vi "LabVIEW.Service.JSON_Input.vi"(4 "Value 4":string="\"Test\"", 6 "Value 3":string="\"Test\"", 7 "Command":T1, 8 "Fehler (Eingang, kein Fehler)":errorcluster, 9 "Value[]":string[](array[string]), 10 "Value 1":string="\"Test\"", 11 "Value 2":string="\"Test\"") -> (0 "Fehler (Ausgang)":errorcluster, 3 "<JSON>":string)   [LabVIEW 2026]
uses:
  LabVIEW.Type Definitions/LabVIEW.Service.JSON_Input_Command.ctl
  <vilib>/JDP Science/JSONtext/support/Format JSON Object.vi
  <vilib>/JDP Science/JSONtext/support/Format JSON Array Text.vi
  <vilib>/JDP Science/JSONtext/JSONtext.lvlib
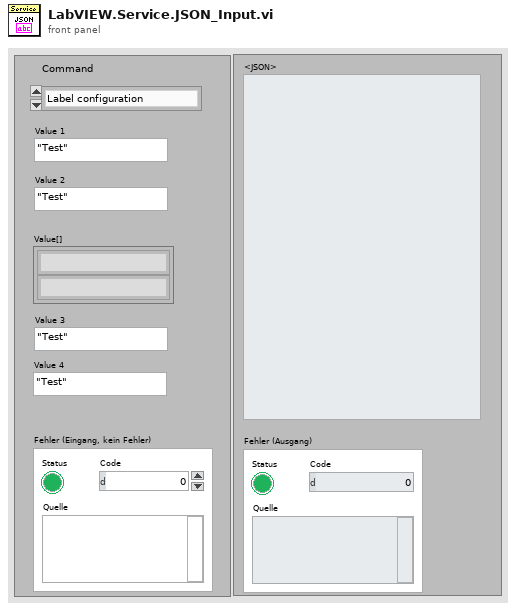
[diagram p1: front panel]
types:
  T1 = typedef "LabVIEW.Service.JSON_Input_Command.ctl" = enum16{"Label configuration", "Label colour ribbon/label tape", "Serial number info text", "Serial number update step", "Serial number bulk lookup", "Vorgang migrate serial numbers to Vorgang", "Vorgang migrate serial numbers to product revision", "Vorgang Update step states", "Fertigmeldung Create/Revert a Fertigmeldung", "User Update a user", "User Update a user role", "Create a new product", "Update a product's data"}
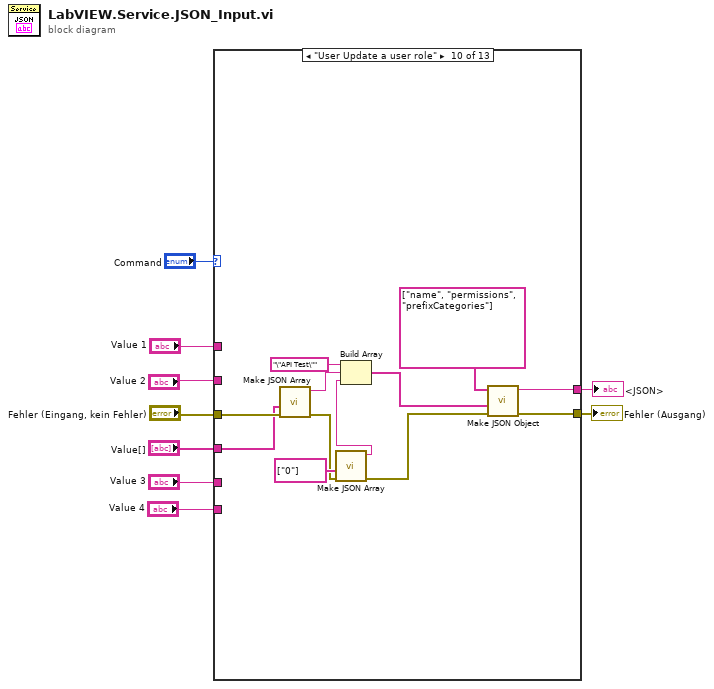
[diagram p0: block diagram]
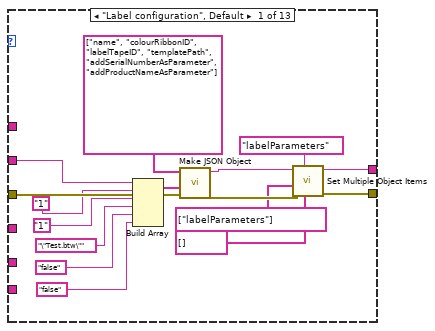
[diagram p2: hidden frame]
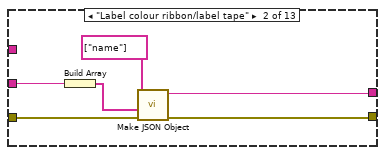
[diagram p3: hidden frame]
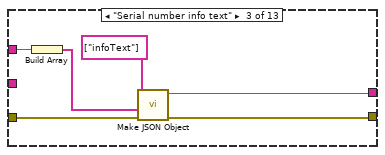
[diagram p4: hidden frame]
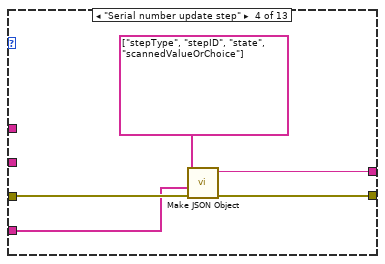
[diagram p5: hidden frame]
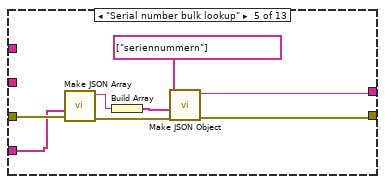
[diagram p6: hidden frame]
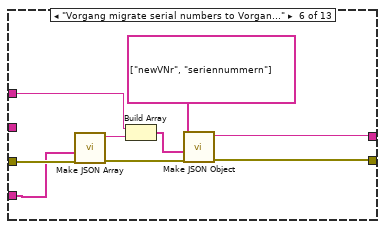
[diagram p7: hidden frame]
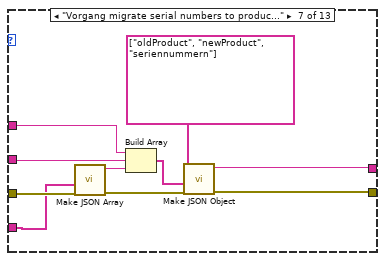
[diagram p8: hidden frame]
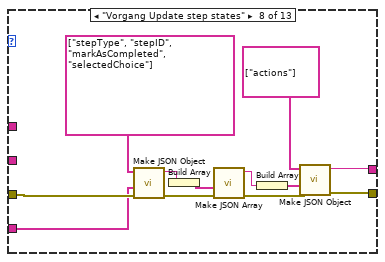
[diagram p9: hidden frame]
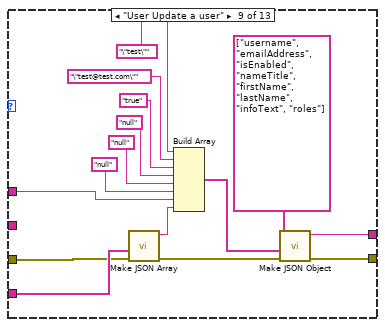
[diagram p10: hidden frame]
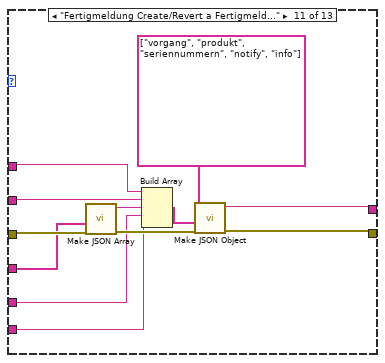
[diagram p11: hidden frame]
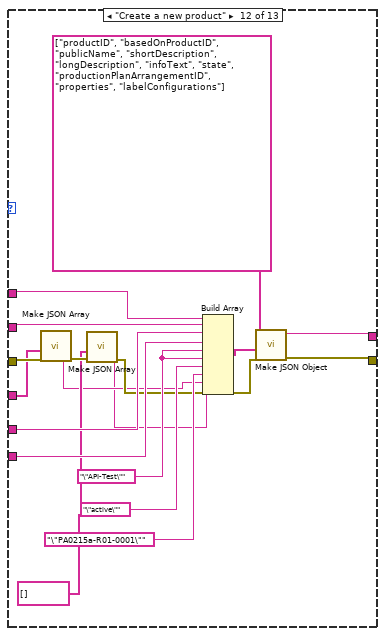
[diagram p12: hidden frame]
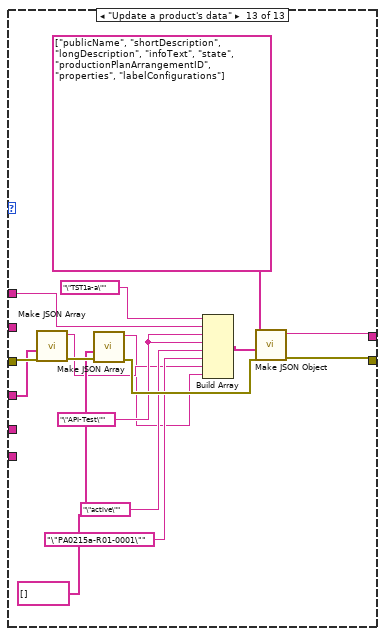
[diagram p13: hidden frame]
diagram:
  n1 = case shown="\"User Update a user role\"" "Command" {
    tunnel: [w25 w26 w33 w38 w46 w54 w64 w77 w93 w107 w112 w132 w150] -> w9
    tunnel: [w24 w29 w35 w40 w49 w53 w63 w78 w94 w108 w111 w131 w149] -> w8
    tunnel: "Fehler (Eingang, kein Fehler)" -> [w16 w30 w36 w41 w45 w55 w65 w79 w86 w105 w116 w136 w152]
    tunnel: "Value 2" -> [w10 w28 _ _ _ _ w60 _ _ _ w114 w134 _]
    tunnel: "Value 1" -> [_ _ w32 _ _ w52 w61 _ w82 _ w115 w135 w144]
    tunnel: "Value[]" -> [_ _ _ w39 w43 w51 w62 w76 w87 w103 w113 w133 w151]
    tunnel: "Value 3" -> [_ _ _ _ _ _ _ _ _ _ w110 w130 _]
    tunnel: "Value 4" -> [_ _ _ _ _ _ _ _ _ _ w109 w129 _]
    frame "Label configuration", Default {
      n2 = Build Array(w10, "1", "1", "\"Test.btw\"", "false", "false") -> (w12:string[])
      n3 = call <vilib>:"Make JSON Object.vi"("error in (no error)"=w16, "JSON Items"=w12, "Item Names"=string[] ["name", "colourRibbonID", "labelTapeID", "templatePath", "addSerialNumberAsParameter", "addProductNameAsParameter"]) -> ("error out"=w23:errorcluster, "<JSON>"=w22:string)  [unwired: 7 in]
      n4 = call <vilib>:"Set Multiple Object Items.vi"("Item Names"=string[] [], "$Path or Item Name"="labelParameters", "error in (no error)"=w23, "JSON Items"=string[] ["labelParameters"], "JSON"=w22) -> ("error out"=w24:errorcluster, "<JSON>"=w25:string)  [unwired: 4 in]
    }
    frame "Label colour ribbon/label tape" {
      n5 = Build Array(w28) -> (w27:string[])
      n6 = call <vilib>:"Make JSON Object.vi"("error in (no error)"=w30, "JSON Items"=w27, "Item Names"=string[] ["name"]) -> ("error out"=w29:errorcluster, "<JSON>"=w26:string)  [unwired: 7 in]
    }
    frame "Serial number info text" {
      n7 = Build Array(w32) -> (w34:string[])
      n8 = call <vilib>:"Make JSON Object.vi"("error in (no error)"=w36, "JSON Items"=w34, "Item Names"=string[] ["infoText"]) -> ("error out"=w35:errorcluster, "<JSON>"=w33:string)  [unwired: 7 in]
    }
    frame "Serial number update step" {
      n9 = call <vilib>:"Make JSON Object.vi"("error in (no error)"=w41, "JSON Items"=w39, "Item Names"=string[] ["stepType", "stepID", "state", "scannedValueOrChoice"]) -> ("error out"=w40:errorcluster, "<JSON>"=w38:string)  [unwired: 7 in]
    }
    frame "Serial number bulk lookup" {
      n10 = call <vilib>:"Make JSON Array.vi"("error in (no error)"=w45, "JSON Elements"=w43) -> ("error out"=w44:errorcluster, "<JSON>"=w48:string)  [unwired: 8 in]
      n11 = Build Array(w48) -> (w47:string[])
      n12 = call <vilib>:"Make JSON Object.vi"("error in (no error)"=w44, "JSON Items"=w47, "Item Names"=string[] ["seriennummern"]) -> ("error out"=w49:errorcluster, "<JSON>"=w46:string)  [unwired: 7 in]
    }
    frame "Vorgang migrate serial numbers to Vorgang" {
      n13 = call <vilib>:"Make JSON Array.vi"("error in (no error)"=w55, "JSON Elements"=w51) -> ("error out"=w56:errorcluster, "<JSON>"=w58:string)  [unwired: 8 in]
      n14 = Build Array(w52, w58) -> (w57:string[])
      n15 = call <vilib>:"Make JSON Object.vi"("error in (no error)"=w56, "JSON Items"=w57, "Item Names"=string[] ["newVNr", "seriennummern"]) -> ("error out"=w53:errorcluster, "<JSON>"=w54:string)  [unwired: 7 in]
    }
    frame "Vorgang migrate serial numbers to product revision" {
      n16 = call <vilib>:"Make JSON Array.vi"("error in (no error)"=w65, "JSON Elements"=w62) -> ("error out"=w66:errorcluster, "<JSON>"=w68:string)  [unwired: 8 in]
      n17 = Build Array(w61, w60, w68) -> (w67:string[])
      n18 = call <vilib>:"Make JSON Object.vi"("error in (no error)"=w66, "JSON Items"=w67, "Item Names"=string[] ["oldProduct", "newProduct", "seriennummern"]) -> ("error out"=w63:errorcluster, "<JSON>"=w64:string)  [unwired: 7 in]
    }
    frame "Vorgang Update step states" {
      n19 = call <vilib>:"Make JSON Object.vi"("error in (no error)"=w79, "JSON Items"=w76, "Item Names"=string[] ["stepType", "stepID", "markAsCompleted", "selectedChoice"]) -> ("error out"=w73:errorcluster, "<JSON>"=w75:string)  [unwired: 7 in]
      n20 = Build Array(w75) -> (w74:string[])
      n21 = call <vilib>:"Make JSON Array.vi"("error in (no error)"=w73, "JSON Elements"=w74) -> ("error out"=w70:errorcluster, "<JSON>"=w72:string)  [unwired: 8 in]
      n22 = Build Array(w72) -> (w71:string[])
      n23 = call <vilib>:"Make JSON Object.vi"("error in (no error)"=w70, "JSON Items"=w71, "Item Names"=string[] ["actions"]) -> ("error out"=w78:errorcluster, "<JSON>"=w77:string)  [unwired: 7 in]
    }
    frame "User Update a user" {
      n24 = call <vilib>:"Make JSON Array.vi"("error in (no error)"=w86, "JSON Elements"=w87) -> ("error out"=w85:errorcluster, "<JSON>"=w84:string)  [unwired: 8 in]
      n25 = Build Array("\"test\"", "\"test@test.com\"", "true", "null", "null" ("Element"), "null" ("Element"), w82, w84) -> (w95:string[])
      n26 = call <vilib>:"Make JSON Object.vi"("error in (no error)"=w85, "JSON Items"=w95, "Item Names"=string[] ["username", "emailAddress", "isEnabled", "nameTitle", "firstName", "lastName", "infoText", "roles"]) -> ("error out"=w94:errorcluster, "<JSON>"=w93:string)  [unwired: 7 in]
    }
    frame "User Update a user role" {
      n27 = call <vilib>:"Make JSON Array.vi"("error in (no error)"=w105, "JSON Elements"=w103) -> ("error out"=w98:errorcluster, "<JSON>"=w101:string)  [unwired: 8 in]
      n28 = call <vilib>:"Make JSON Array.vi"("error in (no error)"=w98, "JSON Elements"=string[] ["0"]) -> ("error out"=w97:errorcluster, "<JSON>"=w99:string)  [unwired: 8 in]
      n29 = Build Array("\"API Test\"" ("Element"), w101, w99) -> (w102:string[])
      n30 = call <vilib>:"Make JSON Object.vi"("error in (no error)"=w97, "JSON Items"=w102, "Item Names"=string[] ["name", "permissions", "prefixCategories"]) -> ("error out"=w108:errorcluster, "<JSON>"=w107:string)  [unwired: 7 in]
    }
    frame "Fertigmeldung Create/Revert a Fertigmeldung" {
      n31 = call <vilib>:"Make JSON Array.vi"("error in (no error)"=w116, "JSON Elements"=w113) -> ("error out"=w117:errorcluster, "<JSON>"=w119:string)  [unwired: 8 in]
      n32 = Build Array(w115, w114, w119, w110, w109) -> (w118:string[])
      n33 = call <vilib>:"Make JSON Object.vi"("error in (no error)"=w117, "JSON Items"=w118, "Item Names"=string[] ["vorgang", "produkt", "seriennummern", "notify", "info"]) -> ("error out"=w111:errorcluster, "<JSON>"=w112:string)  [unwired: 7 in]
    }
    frame "Create a new product" {
      w128 = "\"API-Test\"" ("Element")
      n34 = call <vilib>:"Make JSON Array.vi"("error in (no error)"=w136, "JSON Elements"=w133) -> ("error out"=w125:errorcluster, "<JSON>"=w122:string)  [unwired: 8 in]
      n35 = call <vilib>:"Make JSON Array.vi"("error in (no error)"=w125, "JSON Elements"=string[] [] ("Value[]")) -> ("error out"=w123:errorcluster, "<JSON>"=w121:string)  [unwired: 8 in]
      n36 = Build Array(w135, w134, w130, w129, w128, w128, "\"active\"" ("Element"), "\"PA0215a-R01-0001\"" ("Element"), w122, w121) -> (w137:string[])
      n37 = call <vilib>:"Make JSON Object.vi"("error in (no error)"=w123, "JSON Items"=w137, "Item Names"=string[] ["productID", "basedOnProductID", "publicName", "shortDescription", "longDescription", "infoText", "state", "productionPlanArrangementID", "properties", "labelConfigurations"]) -> ("error out"=w131:errorcluster, "<JSON>"=w132:string)  [unwired: 7 in]
    }
    frame "Update a product's data" {
      w143 = "\"API-Test\"" ("Element")
      n38 = call <vilib>:"Make JSON Array.vi"("error in (no error)"=w152, "JSON Elements"=w151) -> ("error out"=w148:errorcluster, "<JSON>"=w140:string)  [unwired: 8 in]
      n39 = call <vilib>:"Make JSON Array.vi"("error in (no error)"=w148, "JSON Elements"=string[] [] ("Value[]")) -> ("error out"=w146:errorcluster, "<JSON>"=w139:string)  [unwired: 8 in]
      n40 = Build Array("\"TST1a-a\"" ("Element"), w144, w143, w143, "\"active\"" ("Element"), "\"PA0215a-R01-0001\"" ("Element"), w140, w139) -> (w153:string[])
      n41 = call <vilib>:"Make JSON Object.vi"("error in (no error)"=w146, "JSON Items"=w153, "Item Names"=string[] ["publicName", "shortDescription", "longDescription", "infoText", "state", "productionPlanArrangementID", "properties", "labelConfigurations"]) -> ("error out"=w149:errorcluster, "<JSON>"=w150:string)  [unwired: 7 in]
    }
  }
  "<JSON>" <- w9
  "Fehler (Ausgang)" <- w8
